vi "Demo 1.vi"() -> ()   [LabVIEW 2026]
panel:
  out "Waveform Chart 2":dbl(graph)
  in  "Numeric 2":dbl
  out "Gauge 2":dbl(knob) scale=0.0..10.0
  out "Waveform Chart":dbl(graph)
  out "Gauge":dbl(knob) scale=0.0..10.0
  in  "Numeric":dbl
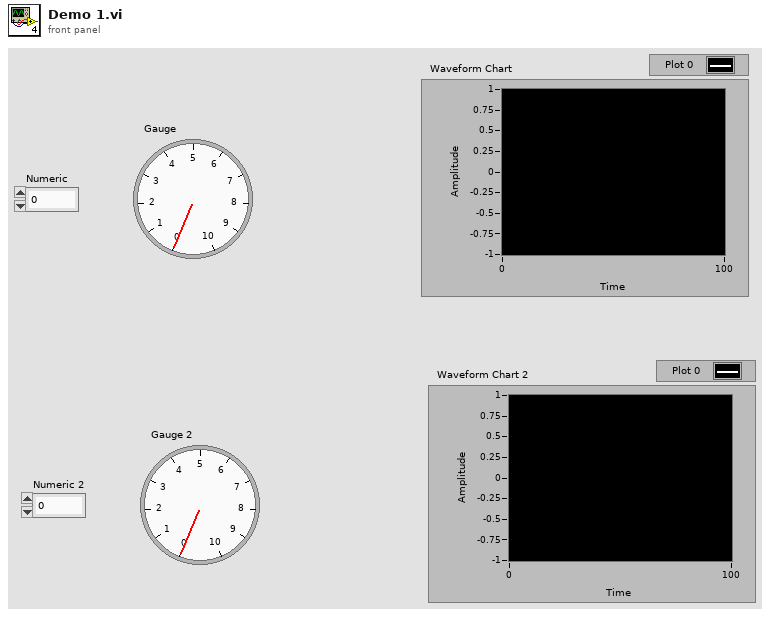
[diagram p1: front panel]
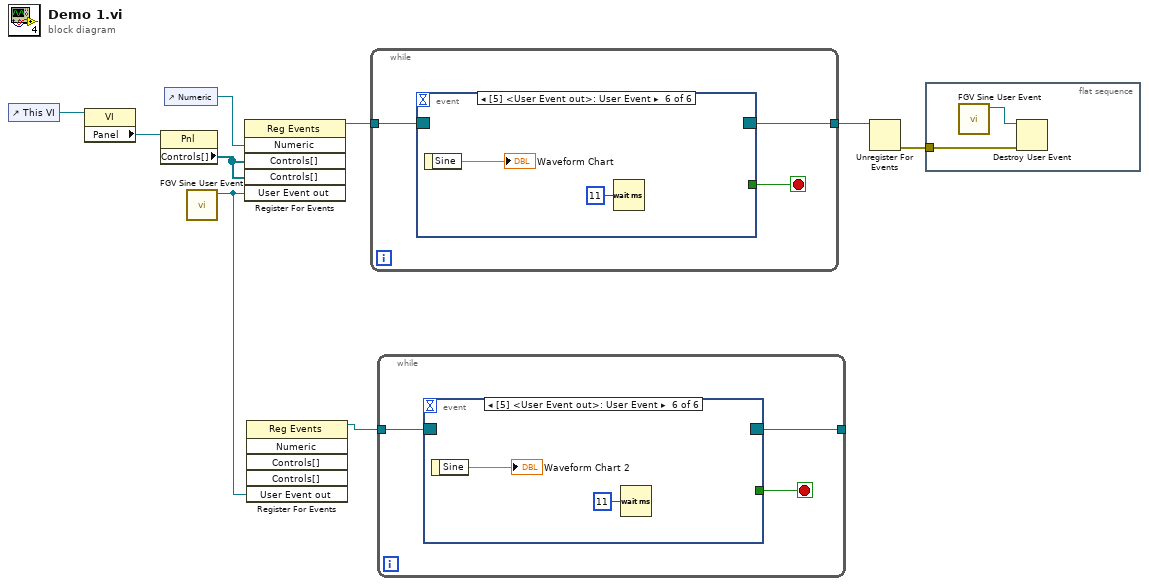
[diagram p0: block diagram]
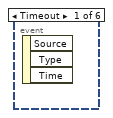
[diagram p2: hidden frame]
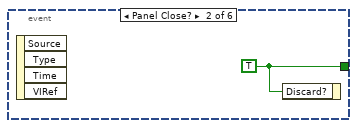
[diagram p3: hidden frame]
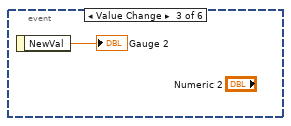
[diagram p4: hidden frame]
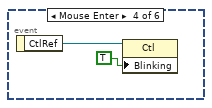
[diagram p5: hidden frame]
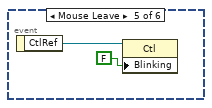
[diagram p6: hidden frame]
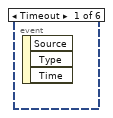
[diagram p7: hidden frame]
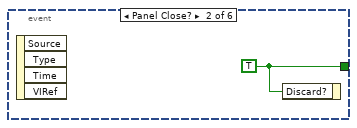
[diagram p8: hidden frame]
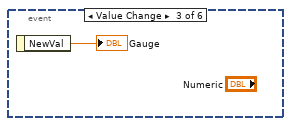
[diagram p9: hidden frame]
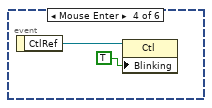
[diagram p10: hidden frame]
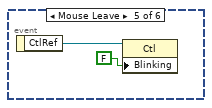
[diagram p11: hidden frame]
diagram:
  n1 = control-ref of="This VI"() -> (w5:refnum<vi>)
  n2 = property class="VI"(reference=w5) -> ("Panel"=w4:refnum<vi>)  [unwired: 1 in, 2 out]
  n3 = property class="Pnl"(reference=w4) -> ("Controls[]"=w3:refnum<vi>[])  [unwired: 1 in, 2 out]
  n4 = control-ref of="Numeric"() -> (w6:refnum<vi>)
  n5 = call "FGV Sine User Event.vi"() -> ("User Event out"=w1:refnum<user-event>)  [unwired: 10 in, 1 out]
  n6 = register-events(w6, w3, w3, w1) -> (reference out=w8:refnum<event-registration>)  [unwired: 2 in, 1 out]
  n7 = register-events(w1) -> (reference out=w2:refnum<event-registration>)  [unwired: 5 in, 1 out]
  n8 = while {
    tunnel: w8 -> [w11]
    tunnel: [w10] -> w7
    stop <- w12 stop-if-true
    n9 = event shown="[5] <User Event out>: User Event" {
      selector: w11 -> [_ _ _ _ _ _]
      dyn-events: [_ _ _ _ _ _] -> w10
      timeout: _ -> [_ _ _ _ _ _]
      tunnel: [_ w13 _ _ _ _] -> w12
      event Timeout {
        n10 = event-data() -> ()  [unwired: 1 in, 3 out]
      }
      event Panel Close? {
        w13 = TRUE ("Discard?")
        n11 = event-data() -> ()  [unwired: 1 in, 4 out]
        n12 = event-data("Discard?"=w13) -> ()  [unwired: 1 in, 1 out]
      }
      event Value Change {
        n13 = event-data() -> ("NewVal"=→"Gauge":dbl)  [unwired: 1 in]
      }
      event Mouse Enter {
        n14 = event-data() -> ("CtlRef"=w16:refnum<vi>)  [unwired: 1 in]
        n15 = property class="Ctl"(reference=w16, "Blinking"=TRUE) -> ()  [unwired: 1 in, 2 out]
      }
      event Mouse Leave {
        n16 = event-data() -> ("CtlRef"=w18:refnum<vi>)  [unwired: 1 in]
        n17 = property class="Ctl"(reference=w18, "Blinking"=FALSE) -> ()  [unwired: 1 in, 2 out]
      }
      event User Event {
        n18 = event-data() -> ("Sine"=→"Waveform Chart":dbl)  [unwired: 1 in]
        n19 = Wait (ms)(milliseconds to wait=u32 11) -> ()  [unwired: 1 out]
      }
    }
  }
  n20 = while {
    tunnel: w2 -> [w22]
    tunnel: [w21] -> _
    stop <- w23 stop-if-true
    n21 = event shown="[5] <User Event out>: User Event" {
      selector: w22 -> [_ _ _ _ _ _]
      dyn-events: [_ _ _ _ _ _] -> w21
      timeout: _ -> [_ _ _ _ _ _]
      tunnel: [_ w24 _ _ _ _] -> w23
      event Timeout {
        n22 = event-data() -> ()  [unwired: 1 in, 3 out]
      }
      event Panel Close? {
        w24 = TRUE ("Discard?")
        n23 = event-data() -> ()  [unwired: 1 in, 4 out]
        n24 = event-data("Discard?"=w24) -> ()  [unwired: 1 in, 1 out]
      }
      event Value Change {
        n25 = event-data() -> ("NewVal"=→"Gauge 2":dbl)  [unwired: 1 in]
      }
      event Mouse Enter {
        n26 = event-data() -> ("CtlRef"=w27:refnum<vi>)  [unwired: 1 in]
        n27 = property class="Ctl"(reference=w27, "Blinking"=TRUE) -> ()  [unwired: 1 in, 2 out]
      }
      event Mouse Leave {
        n28 = event-data() -> ("CtlRef"=w29:refnum<vi>)  [unwired: 1 in]
        n29 = property class="Ctl"(reference=w29, "Blinking"=FALSE) -> ()  [unwired: 1 in, 2 out]
      }
      event User Event {
        n30 = event-data() -> ("Sine"=→"Waveform Chart 2":dbl)  [unwired: 1 in]
        n31 = Wait (ms)(milliseconds to wait=u32 11) -> ()  [unwired: 1 out]
      }
    }
  }
  n32 = Unregister For Events(event registration refnum=w7) -> (error out=w9:errorcluster)  [unwired: 1 in]
  n33 = flat-sequence {
    tunnel: w9 -> [w33]
    frame #0 {
      n34 = call "FGV Sine User Event.vi"() -> ("User Event out"=w32:refnum<user-event>)  [unwired: 10 in, 1 out]
      n35 = Destroy User Event(user event=w32, error in=w33) -> ()  [unwired: 1 out]
    }
  }
